vi "Strings - Create Pseudo Random String.vi"(2 "Length (16)":i32=10) -> (7 "Pseudorandom String":string)   [LabVIEW 2019, in "KoRE-MQTT.lvlib"]
doc: "Copyright (c) 2025 KoRElibs.com\nSPDX-License-Identifier: EUPL-1.2\n\nThis VI is licensed under the European Union Public License (EUPL) Version 1.2. You may use this VI unmodified in proprietary works. If you distribute a modified version of this file, the modified file must be released under the EUPL-1.2. Full license: https://joinup.ec.europa.eu/asset/eupl/eupl/1.2/"
uses:
  KoRE-MQTT.lvlib
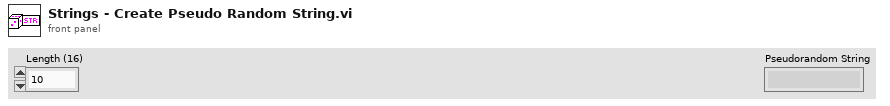
[diagram p1: front panel]
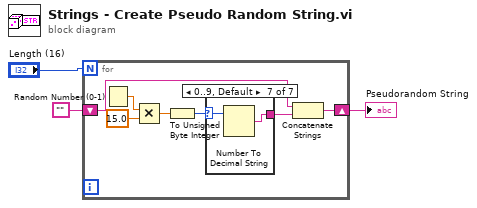
[diagram p0: block diagram]
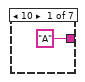
[diagram p2: hidden frame]
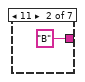
[diagram p3: hidden frame]
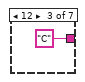
[diagram p4: hidden frame]
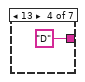
[diagram p5: hidden frame]
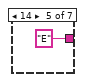
[diagram p6: hidden frame]
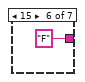
[diagram p7: hidden frame]
diagram:
  n1 = for {
    N: "Length (16)" -> [_]
    shift-right: [w8] -> w1
    shift-left: "" -> [w7]
    n2 = Random Number (0-1)() -> (number: 0 to 1=w4:dbl)
    n3 = Multiply(x=w4, y=15.0) -> (x*y=w6:dbl)
    n4 = To Unsigned Byte Integer(number=w6) -> (unsigned 8bit integer=w5:u8)
    n5 = case shown="0..9, Default" w5 {
      selector: w5 -> [_ _ _ _ _ _ w18]
      tunnel: ["A" "B" "C" "D" "E" "F" w17] -> w9
      frame 10 {
      }
      frame 11 {
      }
      frame 12 {
      }
      frame 13 {
      }
      frame 14 {
      }
      frame 15 {
      }
      frame 0..9, Default {
        n6 = Number To Decimal String(number=w18) -> (decimal integer string=w17:string)  [unwired: 1 in]
      }
    }
    n7 = Concatenate Strings(w7, w9) -> (w8:string)
  }
  "Pseudorandom String" <- w1
